vi "Get a Single Analog Cluster.vi"(10 "Parameter Name":string, 11 "Analog Input List":T1[](array[typedef])) -> (3 "Analog Input Cluster":T1)   [LabVIEW 2021]
uses:
  Analog Cluster.ctl
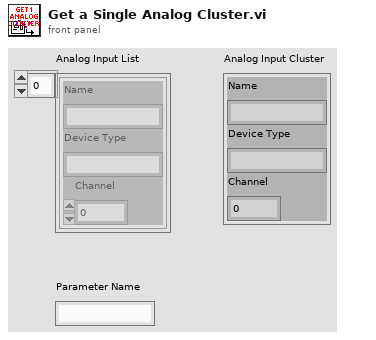
[diagram p1: front panel]
types:
  T1 = typedef "Analog Cluster.ctl" = cluster{"Name":string, "Device Type":string, "Channel":i32}
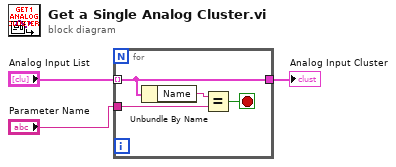
[diagram p0: block diagram]
diagram:
  n1 = for {
    tunnel: "Analog Input List" -> [w6] mode=indexing
    tunnel: "Parameter Name" -> [w7]
    tunnel: [w6] -> w3
    stop <- w5 stop-if-true
    n2 = Unbundle By Name(w6) -> ("Name"=w4:string)
    n3 = Equal?(x=w4, y=w7) -> (x = y?=w5:bool)
  }
  "Analog Input Cluster" <- w3
